vi "str to datetime.vi"(2 "String":string) -> (6 "Time Stamp":timestamp)   [LabVIEW 2014, in "OPCUA XML(dev).lvlib"]
uses:
  OPCUA XML(dev).lvlib
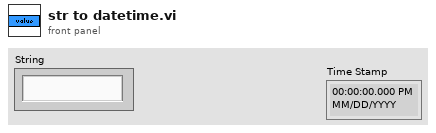
[diagram p1: front panel]
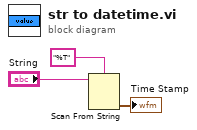
[diagram p0: block diagram]
diagram:
  n1 = Scan From String(format string="%T", input string="String") -> (output 1=→"Time Stamp":timestamp)  [unwired: 3 in, 3 out]
